vi "openbci_channel_count.vi"(8 "error in (no error)":errorcluster, 10 "reset_str_in":string, 11 "OBCI dev in":T1={"COM port"="", "n_ch (8)"=enum."8 Channels", "delay_tx"=50}) -> (0 "error out":errorcluster, 2 "str_out":string, 3 "OBCI dev out":T1={"COM port"="", "n_ch (8)"=enum."8 Channels", "delay_tx"=50})   [LabVIEW 2013]
doc: "Sends a command for 8 or 16 channels to the OpenBCI board"
uses:
  Control Def/openbci_device.ctl
  Control Def/channel_count.ctl
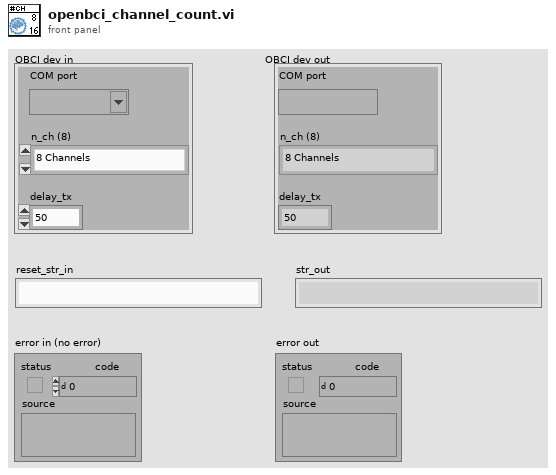
[diagram p1: front panel]
types:
  T1 = typedef "openbci_device.ctl" = cluster{"COM port":refnum<visa-resource-name>, "n_ch (8)":T2, "delay_tx":u32}
  T2 = typedef "channel_count.ctl" = enum16{"8 Channels", "16 Channels"}
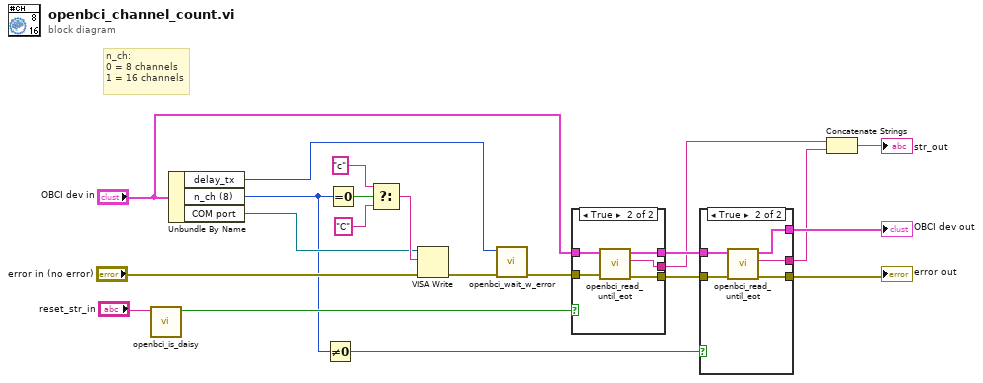
[diagram p0: block diagram]
diagram:
  # "n_ch:\n0 = 8 channels\n1 = 16 channels"
  n1 = call "openbci_is_daisy.vi"("reset_str_in"="reset_str_in") -> ("daisy board?"=w12:bool)  [unwired: 10 in]
  n2 = Unbundle By Name("OBCI dev in") -> ("delay_tx"=w14:u32, "n_ch (8)"=w10:T2, "COM port"=w16:refnum<visa-resource-name>)
  n3 = Not Equal To 0?(x=w10) -> (x != 0?=w9:bool)
  n4 = Equal To 0?(x=w10) -> (x = 0?=w20:bool)
  n5 = Select(t="c", s=w20, f="C") -> (s? t:f=w18:string)
  n6 = VISA Write(VISA resource name=w16, write buffer=w18, error in (no error)="error in (no error)") -> (error out=w15:errorcluster)  [unwired: 2 out]
  n7 = call "openbci_wait_w_error.vi"("error in (no error)"=w15, "milliseconds to wait"=w14) -> ("error out"=w11:errorcluster)  [unwired: 9 in]
  n8 = case shown="True" w12 {
    tunnel: w11 -> [w23 w28]
    tunnel: [w23 w27] -> w8
    tunnel: "OBCI dev in" -> [w22 w26]
    tunnel: [w22 w25] -> w5
    tunnel: [_ w24] -> w3
    frame False {
    }
    frame True {
      n9 = call "openbci_read_until_eot.vi"("error in"=w28, "OBCI dev in"=w26) -> ("error out"=w27:errorcluster, "string"=w24:string, "OBCI dev out"=w25:T1)  [unwired: 7 in]
    }
  }
  n10 = case shown="True" w9 {
    tunnel: w8 -> [w29 w35]
    tunnel: [w29 w34] -> w7
    tunnel: w5 -> [w30 w33]
    tunnel: [w30 w32] -> w4
    tunnel: [_ w31] -> w2
    frame False {
    }
    frame True {
      n11 = call "openbci_read_until_eot.vi"("error in"=w35, "OBCI dev in"=w33) -> ("error out"=w34:errorcluster, "string"=w31:string, "OBCI dev out"=w32:T1)  [unwired: 7 in]
    }
  }
  "error out" <- w7
  "OBCI dev out" <- w4
  n12 = Concatenate Strings(w3, w2) -> (→"str_out":string)
